vi "Main.vi"() -> ()   [LabVIEW 2018, in "StatePatternDemo.lvclass"]
uses:
  StatePatternDemo.lvclass
  Player Class/Player.lvclass
  ConsoleOut/Print Options.ctl
  Player Class/Player.lvclass/Player.ctl
  State Class/State.lvclass
panel:
  out "error out":errorcluster
  in  "Previous Button":bool
  in  "Next Button":bool
  in  "Play Button":bool
  in  "Stop":bool
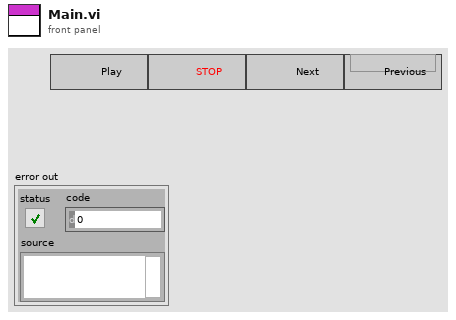
[diagram p1: front panel]
types:
  T1 = typedef "Print Options.ctl" = enum16{"Create", "Get Reference", "Print", "Print Header", "Close"}
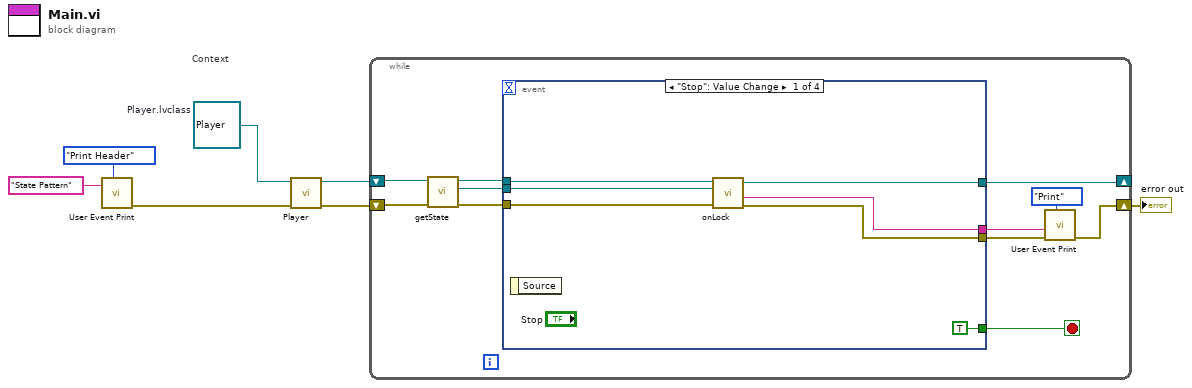
[diagram p0: block diagram]
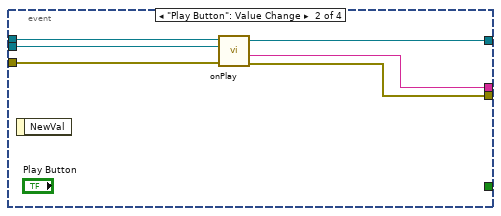
[diagram p2: hidden frame]
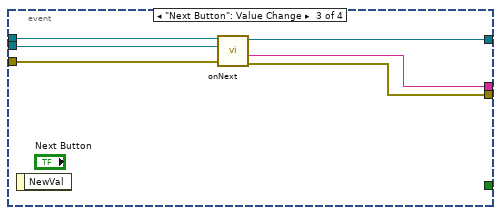
[diagram p3: hidden frame]
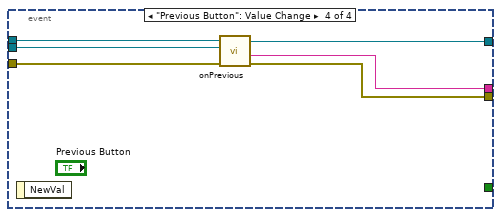
[diagram p4: hidden frame]
diagram:
  w7 = refnum<class "Player.lvclass"> refnum  # Player.lvclass
  # "Context"
  n1 = call "User Event Print.vi"("Options"=Print_Options."Print Header", "String to Print"="State Pattern") -> ("error out"=w4:errorcluster)  [unwired: 8 in, 1 out]
  n2 = call "Player.vi"("error in (no error)"=w4, "Player in"=w7) -> ("error out"=w2:errorcluster, "Player out"=w6:refnum<class "Player.lvclass">)  [unwired: 8 in]
  n3 = while {
    shift-right: [w17] -> _
    shift-left: w6 -> [w8]
    shift-right: [w13] -> w1
    shift-left: w2 -> [w9]
    stop <- w18 stop-if-true
    n4 = call "getState.vi"("error in (no error)"=w9, "Player in"=w8) -> ("error out"=w10:errorcluster, "State.lvclass"=w12:refnum<class "State.lvclass">, "Player out"=w11:refnum<class "Player.lvclass">)  [unwired: 7 in]
    n5 = event shown="[0] \"Stop\": Value Change" {
      selector: _ -> [_ _ _ _]
      dyn-events: _ -> [_ _ _ _]
      timeout: _ -> [_ _ _ _]
      tunnel: [TRUE _ _ _] -> w18
      tunnel: w11 -> [w19 w31 w37 w43]
      tunnel: [w24 w30 w36 w42] -> w17
      tunnel: [w23 w29 w35 w41] -> w16
      tunnel: w10 -> [w20 w28 w34 w40]
      tunnel: [w22 w27 w33 w39] -> w14
      tunnel: w12 -> [w21 w26 w32 w38]
      event "Stop": Value Change {
        n6 = event-data() -> ()  [unwired: 1 in, 1 out]
        n7 = call-dynamic "onLock.vi"("error in (no error)"=w20, "Player In"=w19, "State in"=w21) -> ("error out"=w22:errorcluster, "String"=w23:string, "Player Out"=w24:refnum<class "Player.lvclass">)  [unwired: 5 in, 1 out]
      }
      event "Play Button": Value Change {
        n8 = event-data() -> ()  [unwired: 1 in, 1 out]
        n9 = call-dynamic "onPlay.vi"("error in (no error)"=w28, "Player In"=w31, "State in"=w26) -> ("error out"=w27:errorcluster, "String"=w29:string, "Player Out"=w30:refnum<class "Player.lvclass">)  [unwired: 5 in, 1 out]
      }
      event "Next Button": Value Change {
        n10 = event-data() -> ()  [unwired: 1 in, 1 out]
        n11 = call-dynamic "onNext.vi"("error in (no error)"=w34, "Player In"=w37, "State in"=w32) -> ("error out"=w33:errorcluster, "String"=w35:string, "Player Out"=w36:refnum<class "Player.lvclass">)  [unwired: 5 in, 1 out]
      }
      event "Previous Button": Value Change {
        n12 = event-data() -> ()  [unwired: 1 in, 1 out]
        n13 = call-dynamic "onPrevious.vi"("error in (no error)"=w40, "Player In"=w43, "State in"=w38) -> ("error out"=w39:errorcluster, "String"=w41:string, "Player Out"=w42:refnum<class "Player.lvclass">)  [unwired: 5 in, 1 out]
      }
    }
    n14 = call "User Event Print.vi"("Options"=Print_Options."Print", "error in (no error)"=w14, "String to Print"=w16) -> ("error out"=w13:errorcluster)  [unwired: 7 in, 1 out]
  }
  "error out" <- w1
